vi "Pitch and Roll (SubVI).vi"(5 "Enable Vertical movement":bool, 6 "Control Cluster in":T1 {"Yaw Speed" scale=-1.0..1.0; "Vertical Speed" scale=-1.0..1.0; "Pitch" scale=-1.0..1.0; "Roll" scale=-1.0..1.0}, 8 "pitch offset":dbl=0.15 format="%#_13g", 9 "roll adjust":dbl=1.5 format="%#_13g") -> (3 "Control Cluster out":T1 {"Yaw Speed" scale=-1.0..1.0; "Vertical Speed" scale=-1.0..1.0; "Pitch" scale=-1.0..1.0; "Roll" scale=-1.0..1.0})   [LabVIEW 2014]
uses:
  Resources/Others/Control cluster.ctl
panel:
  in  "vertical speed offset":sgl
  in  "yaw adjust":dbl=2.0
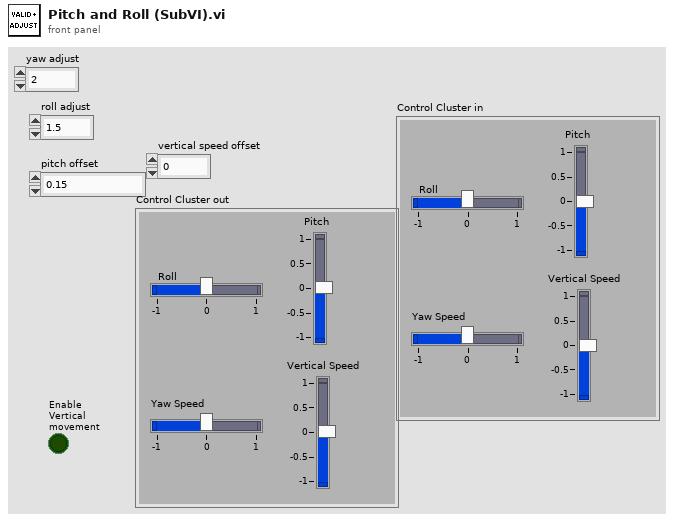
[diagram p1: front panel]
types:
  T1 = typedef "Control cluster.ctl" = cluster{"Roll":sgl, "Pitch":sgl, "Vertical Speed":sgl, "Yaw Speed":sgl}
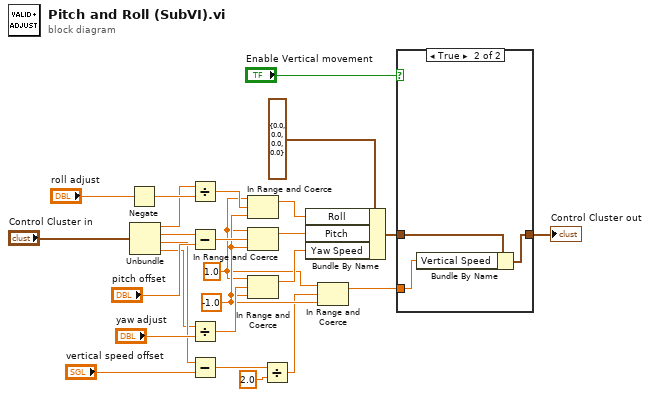
[diagram p0: block diagram]
diagram:
  w17 = -1.0 ("lower limit")
  w16 = 1.0 ("upper limit")
  n1 = Negate(x="roll adjust") -> (-x=w23:dbl)
  n2 = Unbundle("Control Cluster in") -> ("Roll"=w1:sgl, "Pitch"=w2:sgl, "Vertical Speed"=w4:sgl, "Yaw Speed"=w3:sgl)
  n3 = Divide(x=w1, y=w23) -> (x/y=w24:dbl)
  n4 = Subtract(x=w2, y="pitch offset") -> (x-y=w25:dbl)
  n5 = Divide(x=w3, y="yaw adjust") -> (x/y=w19:dbl)
  n6 = Subtract(x=w4, y="vertical speed offset") -> (x-y=w14:sgl)
  n7 = In Range and Coerce(upper limit=w16, x=w24, lower limit=w17) -> (coerced(x)=w26:dbl)  [unwired: 1 out]
  n8 = In Range and Coerce(upper limit=w16, x=w25, lower limit=w17) -> (coerced(x)=w6:dbl)  [unwired: 1 out]
  n9 = In Range and Coerce(upper limit=w16, x=w19, lower limit=w17) -> (coerced(x)=w20:dbl)  [unwired: 1 out]
  n10 = Divide(x=w14, y=sgl 2.0) -> (x/y=w13:sgl)
  n11 = Bundle By Name(cluster=T1 {"Roll"=0.0, "Pitch"=0.0, "Vertical Speed"=0.0, "Yaw Speed"=0.0} ("Control Cluster out"), "Roll"=w26, "Pitch"=w6, "Yaw Speed"=w20) -> (w10:T1)
  n12 = In Range and Coerce(upper limit=w16, x=w13, lower limit=w17) -> (coerced(x)=w7:dbl)  [unwired: 1 out]
  n13 = case shown="True" "Enable Vertical movement" {
    tunnel: w10 -> [w27 w29]
    tunnel: [w27 w28] -> w9
    tunnel: w7 -> [_ w30]
    frame False {
    }
    frame True {
      n14 = Bundle By Name(cluster=w29, "Vertical Speed"=w30) -> (w28:T1)
    }
  }
  "Control Cluster out" <- w9
